vi "filter tags by writer.vi"(10 "module exceptions":string[](array[string]), 11 "engine configuration in":refnum<class "engine configuration.lvclass">) -> (2 "tag list":refnum<class "tag descriptor.lvclass">[](array[class]), 3 "engine configuration out":refnum<class "engine configuration.lvclass">)   [LabVIEW 2014, in "engine configuration.lvclass"]
doc: "Returns a list of tags that don't have a writer unless that writer is contained in the list of 'module exceptions'."
uses:
  engine configuration.lvclass
  <vilib>/NI/Tag Bus/tag/tag descriptor.lvclass
  engine configuration.lvclass/engine configuration.ctl
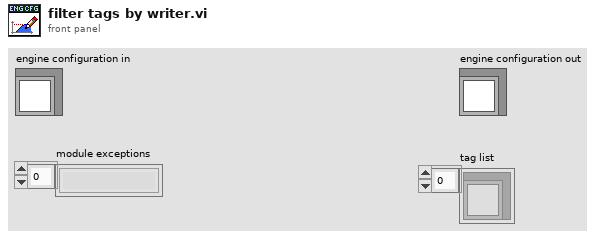
[diagram p1: front panel]
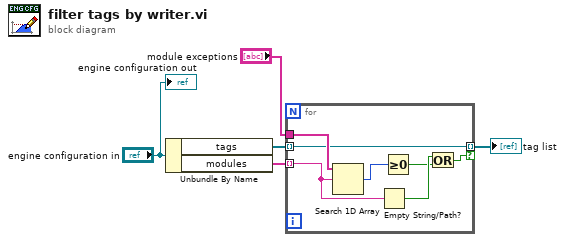
[diagram p0: block diagram]
diagram:
  n1 = Unbundle By Name("engine configuration in") -> ("tags"=w2:refnum<class "tag descriptor.lvclass">[], "modules"=w1:string[])
  n2 = for {
    tunnel: [w7] -> w4 mode=indexing if=w9
    tunnel: "module exceptions" -> [w11]
    tunnel: w2 -> [w7] mode=indexing
    tunnel: w1 -> [w6] mode=indexing
    n3 = Search 1D Array(1D array=w11, element=w6) -> (index of element=w10:i32)  [unwired: 1 in]
    n4 = Empty String/Path?(string/path=w6) -> (empty?=w12:bool)
    n5 = Greater Or Equal To 0?(x=w10) -> (x >= 0?=w8:bool)
    n6 = Or(x=w12, y=w8) -> (x .or. y?=w9:bool)
  }
  "tag list" <- w4
  "engine configuration out" <- "engine configuration in"
